vi "Dispose Report.vi"(0 "report in":refnum<class "ooWriter.lvclass">, 5 "wait until printing completed? (T)":bool=TRUE, 9 "save changes? (F)":bool, 11 "error in (no error)":errorcluster, 12 "close report? (T)":bool=TRUE) -> (15 "error out":errorcluster)   [LabVIEW 2009, in "ooWriter.lvclass"]
doc: "Closes the report and releases its interface, which saves memory."
uses:
  ooWriter.lvclass
  ooWriter.lvclass/ooWriter.ctl
  C:/Projets/LAVAG/OpenOfficeRGT/AODL/DLLs/AODL.dll
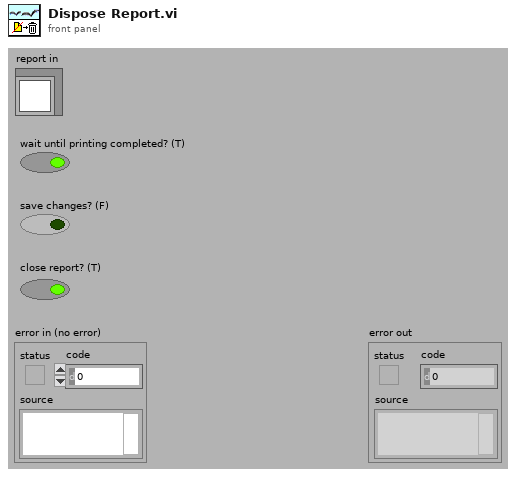
[diagram p1: front panel]
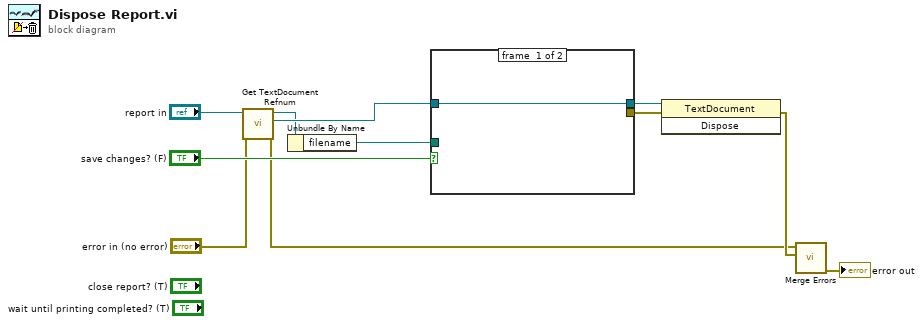
[diagram p0: block diagram]
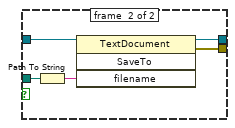
[diagram p2: hidden frame]
diagram:
  n1 = call-dynamic "Get TextDocument Refnum.vi"("error in (no error)"="error in (no error)", "ooWriter in"="report in") -> ("error out"=w2:errorcluster, "TextDocument"=w4:refnum<k24>, "ooWriter out"=w1:refnum<class "ooWriter.lvclass">)  [unwired: 7 in]
  n2 = Unbundle By Name(w1) -> ("filename"=w10:path)
  n3 = case shown="True" "save changes? (F)" {
    tunnel: w4 -> [w12 w17]
    tunnel: [w12 w16] -> w9
    tunnel: w10 -> [_ w15]
    tunnel: [_ w13] -> w8
    frame #0 {
    }
    frame #1 {
      n4 = Path To String(path=w15) -> (string=w14:string)
      n5 = invoke class="TextDocument" method="SaveTo"(reference=w17, "filename"=w14) -> (reference out=w16:refnum<k24>, error out=w13:errorcluster)  [unwired: 2 in, 2 out]
    }
  }
  n6 = invoke class="TextDocument" method="Dispose"(reference=w9, error in=w8) -> (error out=w7:errorcluster)  [unwired: 1 in, 2 out]
  n7 = call <vilib>:"Merge Errors.vi"("error in 2 (no error)"=w7, "error in 1 (no error)"=w2) -> ("error out"=→"error out":errorcluster)  [unwired: 5 in]
